vi "GV_TC1_M.vi"() -> ()   [LabVIEW 2025]
panel:
  out "TC_Monitor":dbl
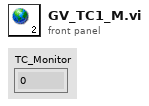
[diagram p1: front panel]
diagram:
